vi "MUX Initialization VI.vi"(8 "error in (no error)":errorcluster, 10 "Custom XML":string, 11 "Device Item Ref in":T1 format="%.0x") -> (0 "error out":errorcluster, 3 "Device Item Ref out":T1 format="%.0x")   [LabVIEW 2013, in "MUX Custom Device.lvlib"]
uses:
  MUX Custom Device.lvlib
  <vilib>/NI Veristand/Custom Device API/Custom Device Item Ref.ctl
  <instrlib>/niSwitch/niSwitch.LLB/niSwitch Topologies.ctl
  MUX Global.vi
  <vilib>/NI Veristand/Custom Device API/Set Item Property (String).vi
  <vilib>/NI Veristand/Custom Device API/Custom Device API.lvlib
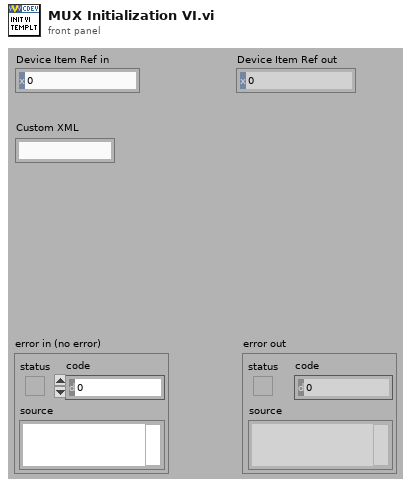
[diagram p1: front panel]
types:
  T1 = typedef "Custom Device API.lvlib/Custom Device Item Ref.ctl" = u64
  T2 = typedef "niSwitch Topologies.ctl" = string
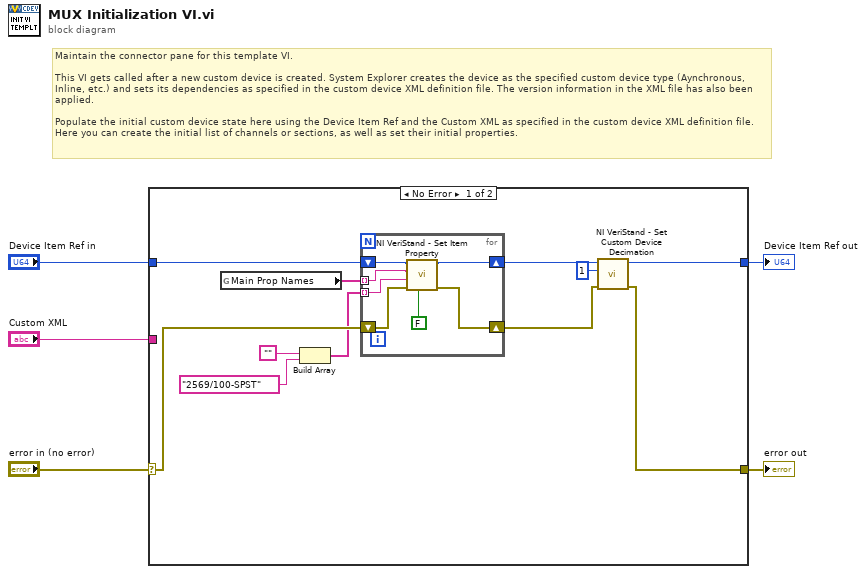
[diagram p0: block diagram]
diagram:
  # "Maintain the connector pane for this template VI.\n\nThis VI gets called after a new custom device is created. System Explorer creates the device as the specified custom device type (Aynchronous, Inline, etc.) and sets its dependencies as specified in the custom device XML definition file. The version information in the XML file has also been applied.\n\nPopulate the initial custom device state here using the Device Item Ref and the Custom XML as specified in the custom device XML definition file. Here you can create the initial list of channels or sections, as well as set their initial properties."
  n1 = case shown="No Error" "error in (no error)" {
    selector: "error in (no error)" -> [w14 w25]
    tunnel: [w9 w25] -> w5
    tunnel: [w8 w24] -> w3
    tunnel: "Device Item Ref in" -> [w16 w24]
    tunnel: "Custom XML" -> [_ _]
    frame No Error {
      n2 = global read "MUX Global.vi" "Main Prop Names"() -> (w15:string[])
      n3 = Build Array("", T2 "2569/100-SPST" ("topology name")) -> (w12:T2[])
      n4 = for {
        tunnel: w15 -> [w20] mode=indexing
        shift-right: [w17] -> w11
        shift-left: w14 -> [w18]
        shift-right: [w21] -> w10
        shift-left: w16 -> [w22]
        tunnel: w12 -> [w19] mode=indexing
        n5 = call-poly <vilib>:"NI VeriStand - Set Item Property.vi"("Binary String (T)"=FALSE, "error in (no error)"=w18, "Value"=w19, "Property Name"=w20, "Item Ref in"=w22) -> ("error out"=w17:errorcluster, "Item Ref out"=w21:T1)  [unwired: 4 in, 1 out]
      }
      n6 = call <vilib>:"NI VeriStand - Set Custom Device Decimation.vi"("error in (no error)"=w11, "Decimation"=1, "Device Ref in"=w10) -> ("error out"=w9:errorcluster, "Device Ref out"=w8:T1)  [unwired: 7 in]
    }
    frame Error {
    }
  }
  "error out" <- w5
  "Device Item Ref out" <- w3
